vi "test - #104.vi"(8 "error in (no error)":errorcluster, 11 "TestCase in":refnum<class "testcase-Supported-Datatype.lvclass">) -> (0 "error out":errorcluster, 3 "TestCase out":refnum<class "testcase-Supported-Datatype.lvclass">)   [LabVIEW 2017, in "testcase-Supported-Datatype.lvclass"]
uses:
  testcase-Supported-Datatype.lvclass
  <vilib>/addons/_JKI Toolkits/VI Tester/TestCase.llb/TestCase.lvclass
  addons/API-String-Arugments-Support/API String Arguments Support.lvlib
  C:/Program Files (x86)/National Instruments/LabVIEW 2017/vi.lib/addons/_JKI Toolkits/VI Tester/TestCase.llb/TestCase.lvclass
panel:
  out "data 3":enum16{"MMMM", "nnnnzzzz", "nnnn", "ZZZZZZZ"}(ring)
  out "error out 3":errorcluster
  out "error out 2":errorcluster
  out "data 2":enum16{"MMMM", "nnnn", "ZZZZZZZ"}(ring)
  out "data":enum16{"1 - MMMM", "2 - nnnnn", "555 - QQQQQ"}(ring)
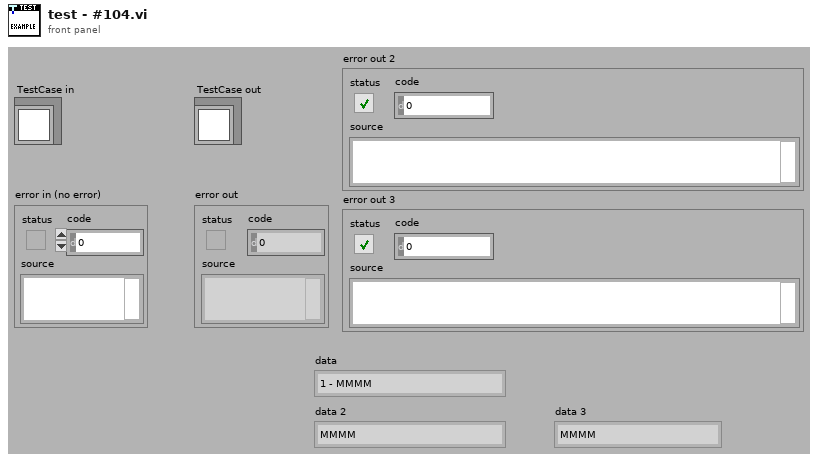
[diagram p1: front panel]
types:
  T1 = enum16{"MMMM", "nnnnzzzz", "nnnn", "ZZZZZZZ", ""}
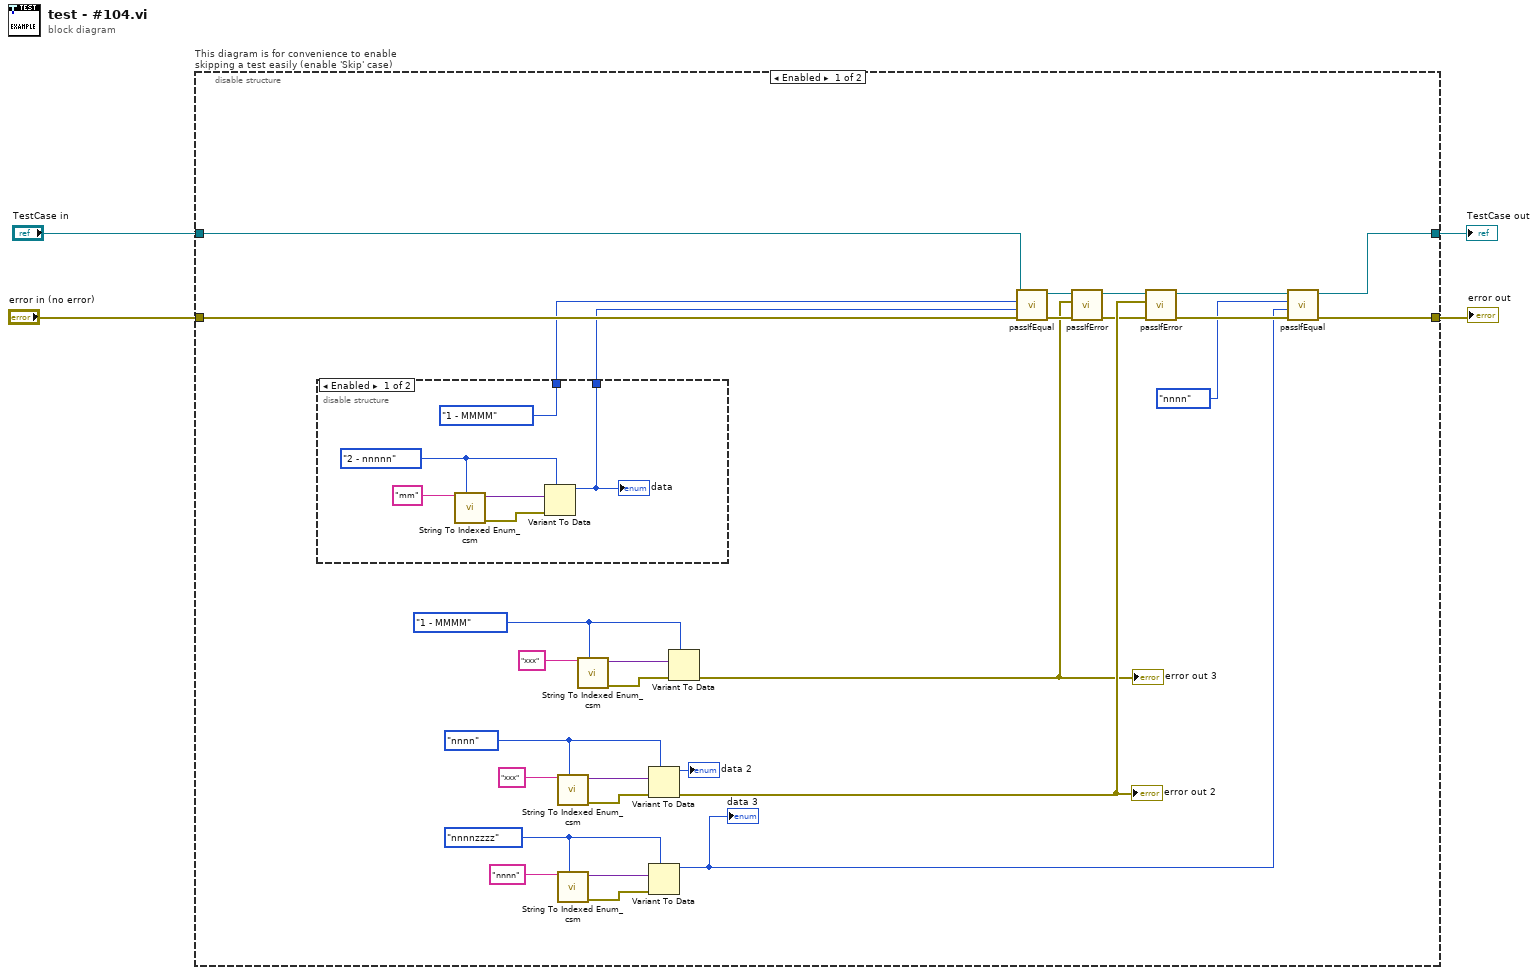
[diagram p0: block diagram]
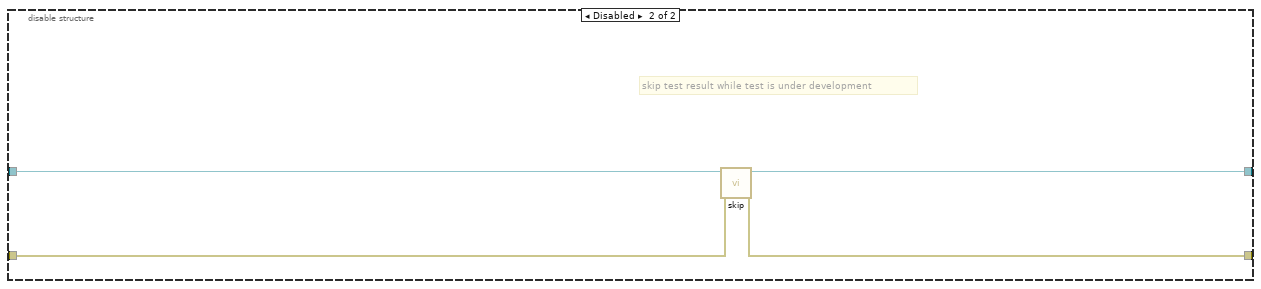
[diagram p3: hidden frame]
diagram:
  n1 = disable-structure "This diagram is for convenience to enable skipping a test easily (enable 'Skip' case)" shown="Enabled" {
    disable-tunnel: "TestCase in" -> [w33 w43]
    disable-tunnel: [w8 w41] -> w1
    disable-tunnel: [w7 w42] -> w3
    disable-tunnel: "error in (no error)" -> [w32 w40]
    frame Enabled {
      w11 = T1."nnnnzzzz" ("Data 6")
      w20 = enum16{"1 - MMMM", "2 - nnnnn", "555 - QQQQQ"}."1 - MMMM" ("Data 6")
      w29 = enum16{"MMMM", "nnnn", "ZZZZZZZ"}."nnnn" ("Data 6")
      n2 = disable-structure shown="Enabled" {
        disable-tunnel: [w35 _] -> w31
        disable-tunnel: [enum16{"1 - MMMM", "2 - nnnnn", "555 - QQQQQ"}."1 - MMMM" ("Data 6") _] -> w30
        frame Enabled {
          w36 = enum16{"1 - MMMM", "2 - nnnnn", "555 - QQQQQ"}."2 - nnnnn" ("Data 6")
          n3 = call "String To Indexed Enum_csm.vi"("Variant"=w36, "String"="mm") -> ("error out"=w37:errorcluster, "Enum"=w38:variant)  [unwired: 8 in]
          n4 = Variant To Data(error in=w37, type=w36, Variant=w38) -> (data=w35:enum16{"1 - MMMM", "2 - nnnnn", "555 - QQQQQ"})  [unwired: 1 out]
          "data" <- w35
        }
        frame Disabled {
        }
      }
      n5 = call "String To Indexed Enum_csm.vi"("Variant"=w29, "String"="xxx") -> ("error out"=w28:errorcluster, "Enum"=w27:variant)  [unwired: 8 in]
      n6 = call "String To Indexed Enum_csm.vi"("Variant"=w11, "String"="nnnn") -> ("error out"=w12:errorcluster, "Enum"=w13:variant)  [unwired: 8 in]
      n7 = call "String To Indexed Enum_csm.vi"("Variant"=w20, "String"="xxx") -> ("error out"=w21:errorcluster, "Enum"=w22:variant)  [unwired: 8 in]
      n8 = Variant To Data(error in=w28, type=w29, Variant=w27) -> (data=→"data 2":enum16{"MMMM", "nnnn", "ZZZZZZZ"}, error out=w25:errorcluster)
      "error out 2" <- w25
      n9 = Variant To Data(error in=w12, type=w11, Variant=w13) -> (data=w6:T1)  [unwired: 1 out]
      "data 3" <- w6
      n10 = Variant To Data(error in=w21, type=w20, Variant=w22) -> (error out=w15:errorcluster)  [unwired: 1 out]
      "error out 3" <- w15
      n11 = call-dynamic "passIfEqual.vi"("error in (no error)"=w32, "y"=w31, "x"=w30, "TestCase in"=w33) -> ("error out"=w16:errorcluster, "TestCase out"=w19:refnum<class "testcase-Supported-Datatype.lvclass">)  [unwired: 6 in]
      n12 = call-dynamic "passIfError.vi"("error in (no error)"=w16, "error"=w15, "TestCase in"=w19) -> ("error out"=w17:errorcluster, "TestCase out"=w18:refnum<class "testcase-Supported-Datatype.lvclass">)  [unwired: 7 in]
      n13 = call-dynamic "passIfError.vi"("error in (no error)"=w17, "error"=w25, "TestCase in"=w18) -> ("error out"=w10:errorcluster, "TestCase out"=w9:refnum<class "testcase-Supported-Datatype.lvclass">)  [unwired: 7 in]
      n14 = call-dynamic "passIfEqual.vi"("error in (no error)"=w10, "y"=w6, "x"=T1."nnnn" ("Data 6"), "TestCase in"=w9) -> ("error out"=w7:errorcluster, "TestCase out"=w8:refnum<class "testcase-Supported-Datatype.lvclass">)  [unwired: 6 in]
    }
    frame Disabled {
      # "skip test result while test is under development"
      n15 = call <vilib>:"skip.vi"("error in (no error)"=w40, "TestCase in"=w43) -> ("error out"=w42:errorcluster, "TestCase out"=w41:refnum<class "testcase-Supported-Datatype.lvclass">)  [unwired: 8 in]
    }
  }
  "error out" <- w3
  "TestCase out" <- w1
